vi "lvmcp_connect.vi"() -> ()   [LabVIEW 2026]
panel:
  out "error out":errorcluster
  in  "other":refnum<vi>
  in  "reference":refnum<vi>
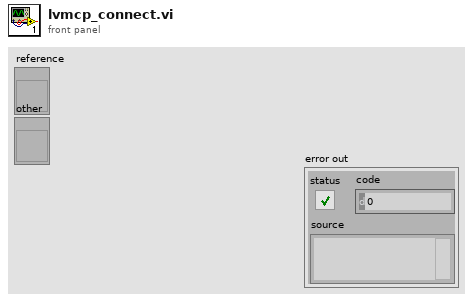
[diagram p1: front panel]
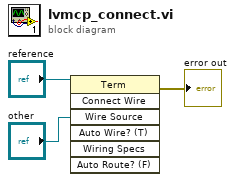
[diagram p0: block diagram]
diagram:
  n1 = invoke class="Term" method="Connect Wire"(reference="reference", "Wire Source"="other") -> (error out=→"error out":errorcluster)  [unwired: 5 in, 6 out]
